vi "ReadChannelsNames.vi"(8 "error in (no error)":errorcluster, 11 "ChannelManagerUI in":refnum<class "ChannelManagerUI.lvclass">) -> (0 "error out":errorcluster, 2 "Channel Names":string[](array[string]), 3 "ChannelManagerUI out":refnum<class "ChannelManagerUI.lvclass">)   [LabVIEW 2021, in "Channel.lvlib" / "ChannelManagerUI.lvlib" / "ChannelManagerUI.lvclass"]
uses:
  ChannelManagerUI.lvclass
  ChannelManagerUI.lvclass/ChannelManagerUI.ctl
  ChannelsManager/ChannelsManager/ChannelsManager.lvclass
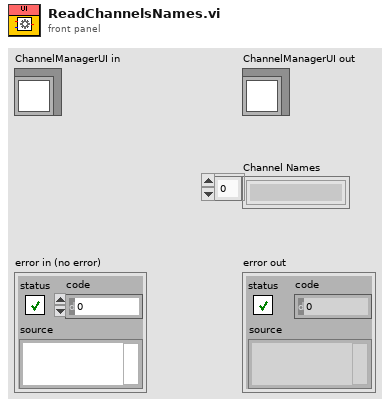
[diagram p1: front panel]
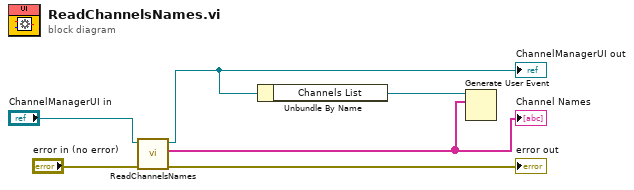
[diagram p0: block diagram]
diagram:
  n1 = call-parent "ReadChannelsNames.vi"("error in (no error)"="error in (no error)", "ChannelsManager in"="ChannelManagerUI in") -> ("error out"=→"error out":errorcluster, "Channel Names"=w1:string[], "ChannelsManager out"=w3:refnum<class "ChannelManagerUI.lvclass">)  [unwired: 7 in]
  "ChannelManagerUI out" <- w3
  "Channel Names" <- w1
  n2 = Unbundle By Name(w3) -> ("Channels List"=w2:refnum<user-event>)
  n3 = Generate User Event(user event=w2, event data cluster=w1) -> ()  [unwired: 2 in, 2 out]
